vi "Connection Handler Worker.vi"(9 "Additional Data":variant, 10 "connection ID":T1, 11 "TCP Server Refnum":refnum<class "JKI TCP Server.lvclass">) -> ()   [LabVIEW 2020, in "CSM-TCP-Router.lvlib"]
uses:
  CSM-TCP-Router.lvlib
  <vilib>/addons/_JKI.lib/_JKI_lib_TCP_Server.llb/TCP Server Connection Session ID Cluster.ctl
  <vilib>/addons/_JKI.lib/_JKI_lib_TCP_Server.llb/JKI TCP Server.lvclass
  tcp-msg type.ctl
  <userlib>/_NEVSTOP/Communicable State Machine(CSM)/AdvanceAPI/CSM - Broadcast Message Type.ctl
  20ff867f-262a-4864-b042-c50abd455195.vi
  9f8653f6-ccbf-4dca-88e7-a4c531b7661f.vi
  bd168d05-2ccd-4f69-90c9-be1b4e621865.vi
  316abe05-dd11-44a4-98b3-32ea1594dc48.vi
  a7f8194b-54d4-448d-8a65-d0b66a8fd47c.vi
  8a9da1d4-9237-4126-a3a1-8a9d876b672d.vi
  66683ee4-8938-4a2b-95b9-1d8ed72716c9.vi
  <userlib>/_NEVSTOP/Communicable State Machine(CSM)/_Support/ChangeFlag/FlagInstance-CSMQ FGV.vi
  <userlib>/_NEVSTOP/Communicable State Machine(CSM)/_Support/ChangeFlag/FlagInstance-Broadcast Cache.vi
  <userlib>/_NEVSTOP/Communicable State Machine(CSM)/AdvanceAPI/CSM - Revert Arguments-Safe String.vi
  <userlib>/_NEVSTOP/Communicable State Machine(CSM)/AdvanceAPI/CSM - Make String Arguments Safe.vi
  <userlib>/_NEVSTOP/Communicable State Machine(CSM)/AdvanceAPI/CSM - Compact Multiple States.vi
  <userlib>/_NEVSTOP/Communicable State Machine(CSM)/_Support/ChangeFlag/ChangeFlag-Read.vi
  <userlib>/_NEVSTOP/Communicable State Machine(CSM)/AdvanceAPI/CSM - Keywords.vi
  <userlib>/_NEVSTOP/Communicable State Machine(CSM)/addons/API-String-Arugments-Support/_Support/Data To API String Arguments.vi
  <userlib>/_NEVSTOP/Communicable State Machine(CSM)/_Support/ChangeFlag/ChangeFlagDB.vi
  <userlib>/_NEVSTOP/Communicable State Machine(CSM)/_Support/BroadcastRegistry/HelperVI/Broadcast Item Key.vi
  <userlib>/_NEVSTOP/Communicable State Machine(CSM)/_Support/FGV-BroadcastRegistry/FGV-BroadcastRegistry(lvlibp).vi
  <userlib>/_NEVSTOP/Communicable State Machine(CSM)/addons/API-String-Arugments-Support/_Support/Query Data as API String Arguments(variant).vi
  <userlib>/_NEVSTOP/Communicable State Machine(CSM)/addons/API-String-Arugments-Support/_Support/Convert API String Arguments to Data(variant).vi
  <userlib>/_NEVSTOP/Communicable State Machine(CSM)/Communicable State Machine.lvlib
  <userlib>/_NEVSTOP/Communicable State Machine(CSM)/_csmHelper/API with lvcsm Support/CSM-Helper API with lvcsm Support.lvlib
  <userlib>/_NEVSTOP/Communicable State Machine(CSM)/_Shared/CSM Shared.lvlib
panel:
  out "State History":string
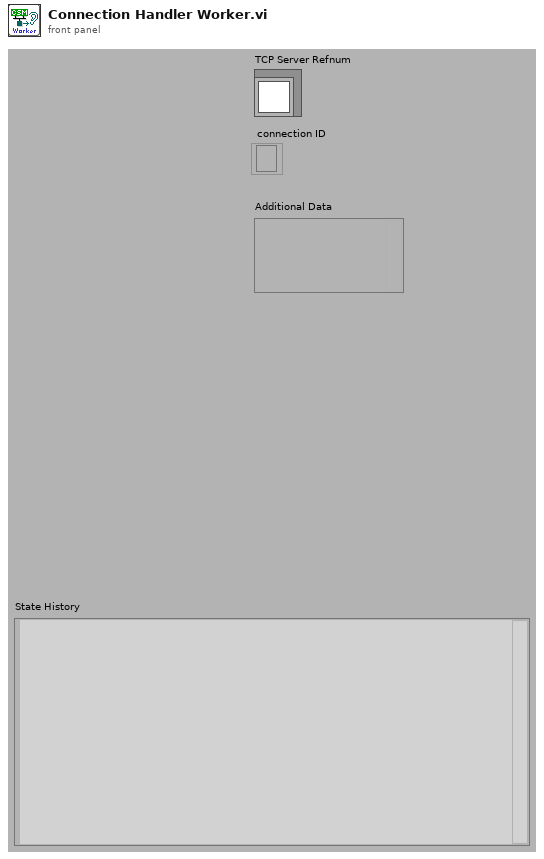
[diagram p1: front panel]
types:
  T1 = typedef "JKI TCP Server.lvclass/TCP Server Connection Session ID Cluster.ctl" = refnum<k5>
  T2 = typedef "CSM-TCP-Router.lvlib/tcp-msg type.ctl" = enum8{"info", "error", "cmd", "cmd-resp", "resp", "async-resp", "status", "interrupt"}
  T3 = typedef "Communicable State Machine.lvlib/CSM - Broadcast Message Type.ctl" = enum16{"<Null>", "Status", "Interrupt"}
  T4 = enum32{"Invalid", "Standard", "Closed", "Hidden", "Minimized", "Maximized"}
  T5 = enum32{"invalid app kind", "Development System", "Run Time System", "Student Edition", "Embedded LabVIEW", "Evaluation", "Custom"}
  T6 = typedef "Communicable State Machine.lvlib/_CSM_Response Source Message.ctl" = cluster{"‘State":string, "’Arguments":string, "’Error":errorcluster}
  T7 = cluster{"Target CSM":string, "Target State":string, "Register Type":T3}[]
  T8 = cluster{"Current VI Reference":refnum<vi>, "Close Panel on Exit?":bool}
  T9 = cluster{"Core":cluster{"Current VI Reference":refnum<vi>, "Close Panel on Exit?":bool}, "Your Boolean data":bool}
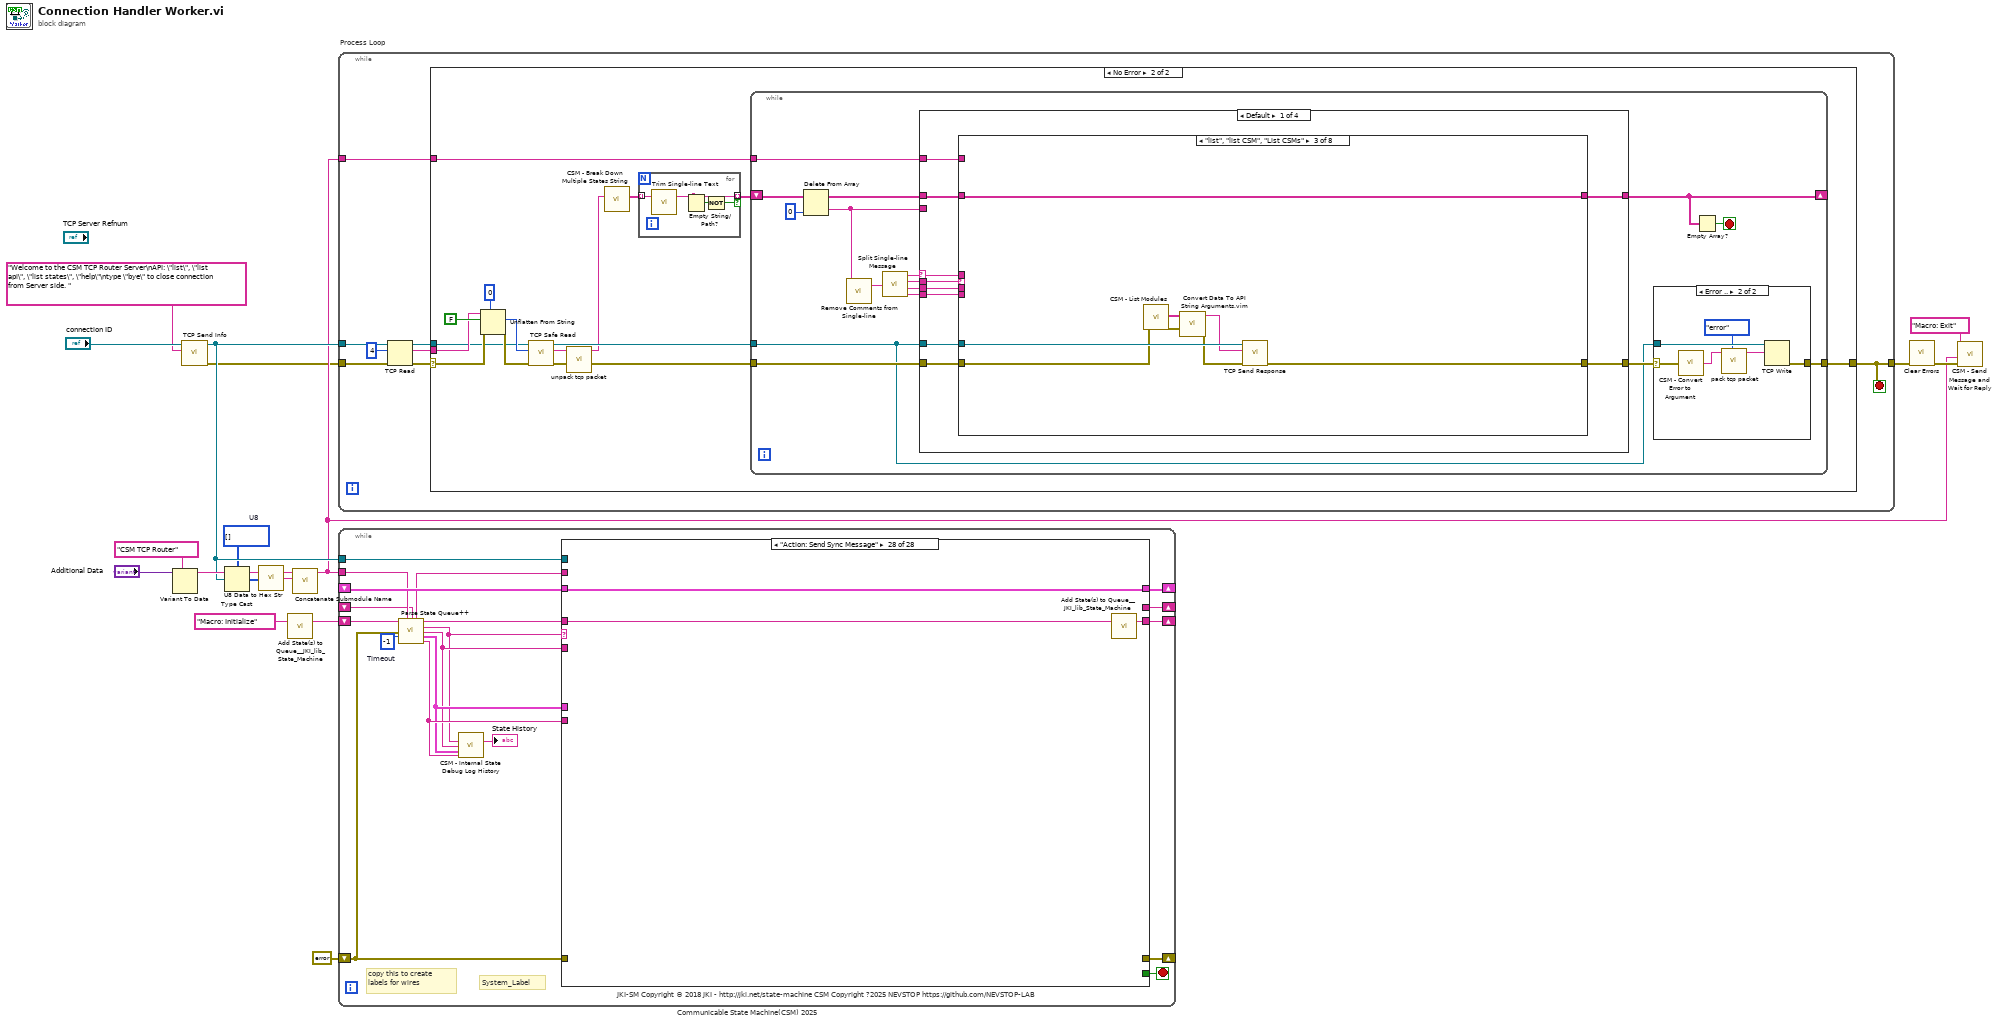
[diagram p0: block diagram]
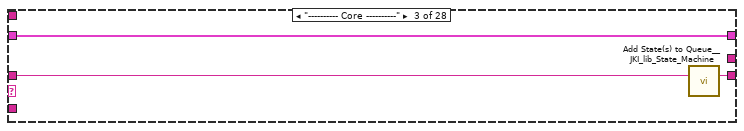
[diagram p4: hidden frame]
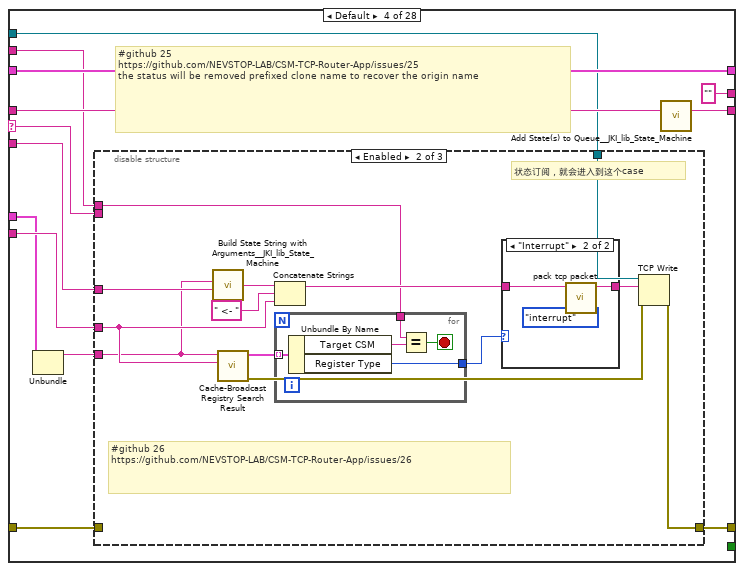
[diagram p5: hidden frame]
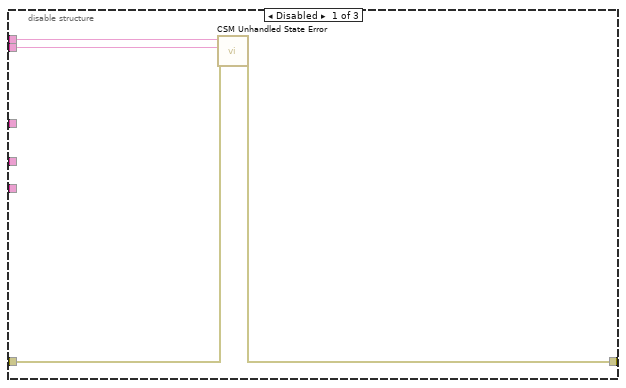
[diagram p6: hidden frame]
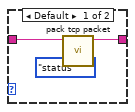
[diagram p7: hidden frame]
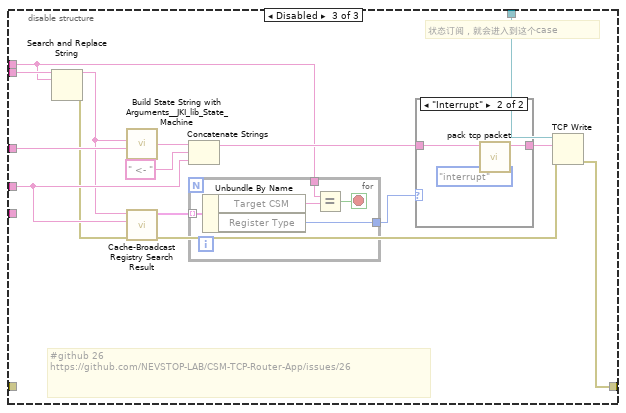
[diagram p8: hidden frame]
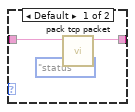
[diagram p9: hidden frame]
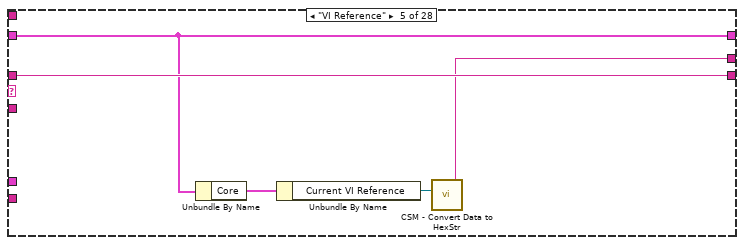
[diagram p10: hidden frame]
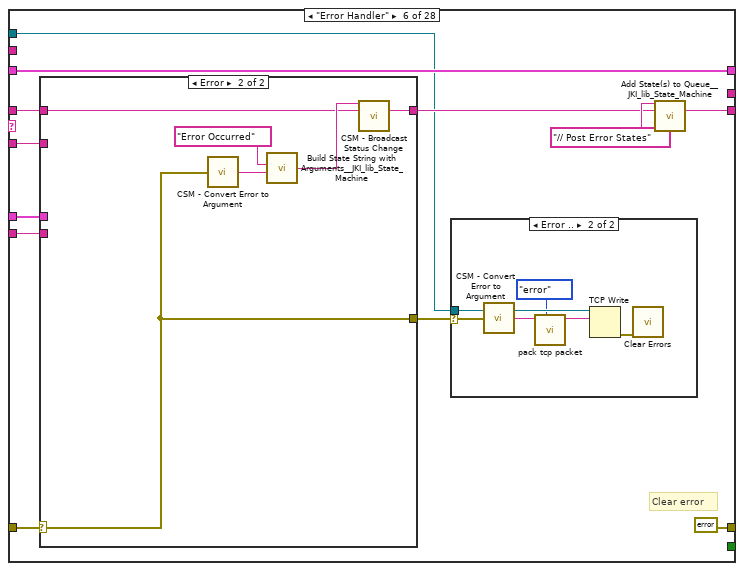
[diagram p11: hidden frame]
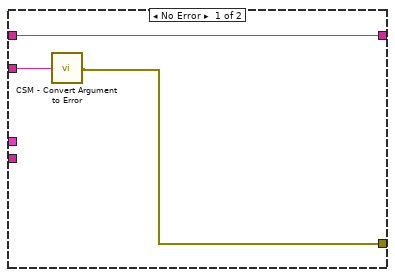
[diagram p13: hidden frame]
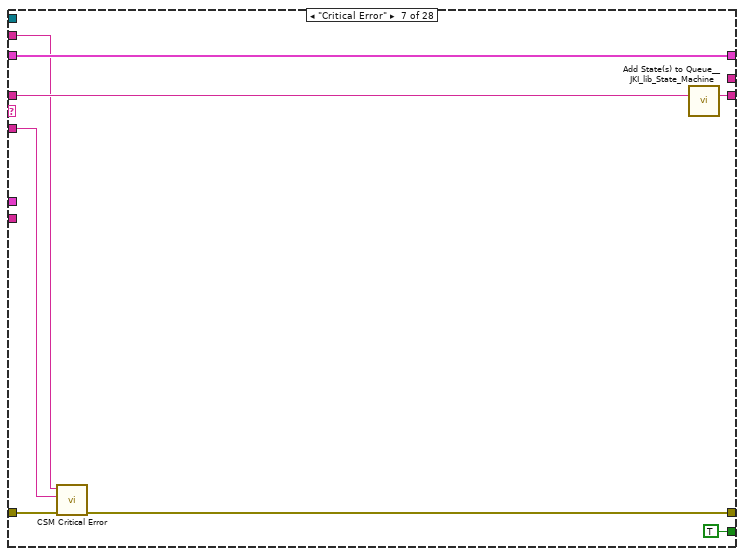
[diagram p14: hidden frame]
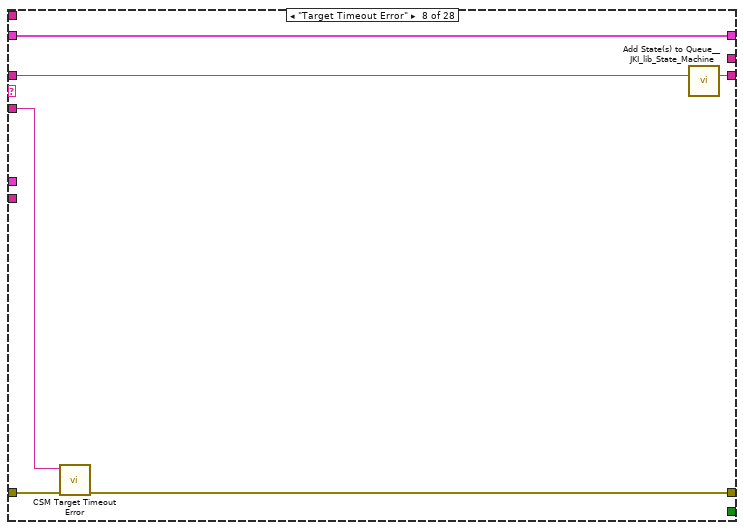
[diagram p15: hidden frame]
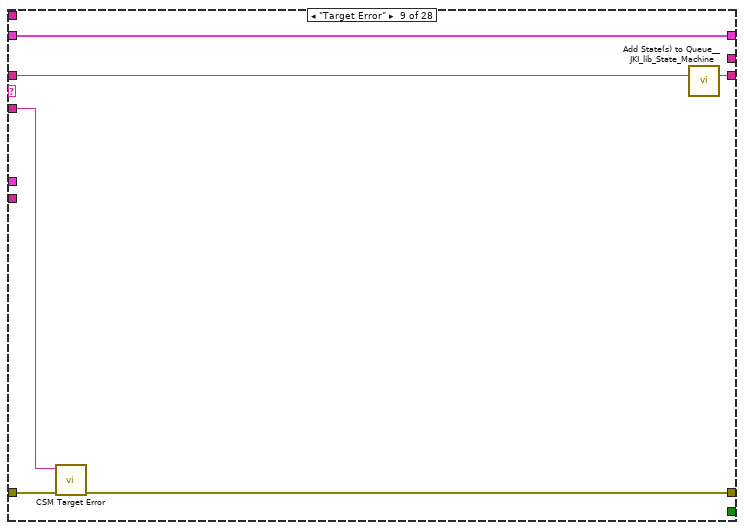
[diagram p16: hidden frame]
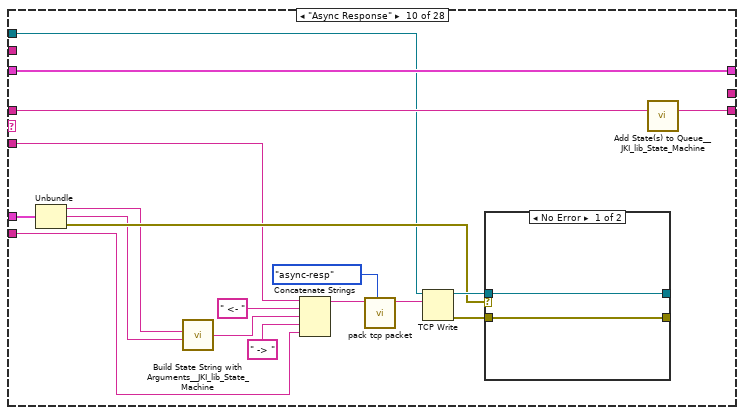
[diagram p17: hidden frame]
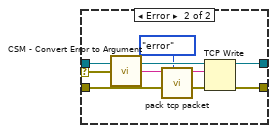
[diagram p18: hidden frame]
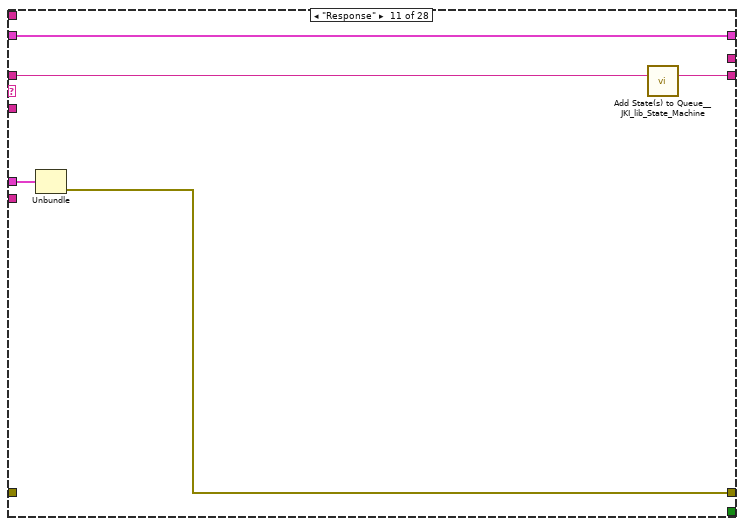
[diagram p19: hidden frame]
diagram:
  w5 = u8[] []  # U8
  n1 = Variant To Data(type="CSM TCP Router" ("Name(\"\" to use uuid)"), Variant="Additional Data") -> (data=w9:string)  [unwired: 1 in, 1 out]
  n2 = call "TCP Send Info.vi"("data in"="Welcome to the CSM TCP Router Server\nAPI: \"list\", \"list api\", \"list states\", \"help\"\ntype \"bye\" to close connection from Server side. ", "TCP Network Connection in"="connection ID") -> ("error out"=w2:errorcluster, "TCP Network Connection out"=w7:T1)  [unwired: 8 in]
  n3 = Type Cast(type=w5, x=w7) -> (*(type *) &x=w4:u8[])
  n4 = call <userlib>:"U8 Data to Hex Str.vi"("U8 Data[]"=w4) -> ("HEX String (0-9,A-F)"=w6:string)
  n5 = call <vilib>:"Add State(s) to Queue__JKI_lib_State_Machine.vi"("State(s) in (\"\")"="Macro: Initialize" ("Init States(\"Macro: Initialize\")")) -> ("States Out"=w15:string)  [unwired: 14 in]
  n6 = call <userlib>:"Concatenate Submodule Name.vi"("Module Name"=w6, "Group Name"=w9) -> ("Submodule Name"=w3:string)  [unwired: 9 in]
  n7 = while "Process Loop" {
    tunnel: w7 -> [w25]
    tunnel: [w21] -> w13
    tunnel: w3 -> [w20]
    tunnel: w2 -> [w18]
    stop <- w21 stop-if-true
    n8 = TCP Read(connection ID=w25, bytes to read=4, error in (no error)=w18) -> (connection ID out=w24:T1, data out=w22:string, error out=w23:errorcluster)  [unwired: 2 in]
    n9 = case shown="No Error" w23 {
      selector: w23 -> [w27 w37]
      tunnel: w24 -> [_ w30]
      tunnel: w22 -> [_ w38]
      tunnel: [w26 w44] -> w21
      tunnel: w20 -> [_ w41]
      frame Error {
        n10 = Unbundle By Name(w27) -> ("code"=w28:i32)
        n11 = case shown="56" w28 {
          tunnel: w27 -> [w29 _]
          tunnel: [w29 _] -> w26
          frame 0, Default {
          }
          frame 56 {
          }
        }
      }
      frame No Error {
        n12 = Unflatten From String(type=0, binary string=w38, data includes array or string size? (T)=FALSE, error in (no error)=w37) -> (value=w33:i32, error out=w36:errorcluster)  [unwired: 2 out]
        n13 = call "TCP Safe Read.vi"("error in (no error)"=w36, "bytes to read"=w33, "TCP Network Connection in"=w30) -> ("error out"=w35:errorcluster, "String"=w32:string, "TCP Network Connection out"=w34:refnum<k5>)  [unwired: 6 in]
        n14 = call "unpack tcp packet.vi"("TCP Pack"=w32) -> ("String"=w31:string)  [unwired: 9 in, 1 out]
        n15 = call <userlib>:"CSM - Break Down Multiple States String.vi"("States"=w31) -> ("Multiple States"=w43:string[])  [unwired: 10 in]
        n16 = for {
          tunnel: w43 -> [w48] mode=indexing
          tunnel: [w47] -> w42 mode=indexing if=w45
          n17 = call <userlib>:"Trim Single-line Text.vi"("single-line text"=w48) -> ("trimed text"=w47:string)  [unwired: 2 in]
          n18 = Empty String/Path?(string/path=w47) -> (empty?=w46:bool)
          n19 = Not(x=w46) -> (.not. x?=w45:bool)
        }
        n20 = while {
          tunnel: w34 -> [w51]
          tunnel: w35 -> [w64]
          tunnel: [w52] -> w44
          shift-right: [w54] -> _
          shift-left: w42 -> [w58]
          tunnel: w41 -> [w49]
          stop <- w55 stop-if-true
          n21 = Delete From Array(array=w58, index=0) -> (deleted portion=w50:string, array with subset deleted=w57:string[])  [unwired: 1 in]
          n22 = call <userlib>:"Remove Comments from Single-line.vi"("single-line text"=w50) -> ("single-line text without comments"=w63:string)  [unwired: 2 in]
          n23 = call <userlib>:"Split Single-line Message.vi"("single-line text"=w63) -> ("operator"=w62:string, "state"=w61:string, "args"=w60:string, "source/target"=w59:string)  [unwired: 6 in]
          n24 = case shown="Default" w62 {
            selector: w62 -> [w75 _ _ _]
            tunnel: w51 -> [w81 w192 w196 w267]
            tunnel: [w80 w191 w200 w271] -> w53
            tunnel: w64 -> [w79 w184 w198 w269]
            tunnel: w61 -> [w78 w186 w195 w266]
            tunnel: w60 -> [w77 w185 w194 w265]
            tunnel: w59 -> [w76 w187 w193 w264]
            tunnel: [w74 w189 w199 w270] -> w54
            tunnel: w57 -> [w73 w189 w199 w270]
            tunnel: w50 -> [_ _ _ _]
            tunnel: w49 -> [w72 w188 w197 w268]
            frame Default {
              n25 = case shown="\"list\", \"list CSM\", \"List CSMs\"" w78 {
                selector: w78 -> [w89 _ _ _ _ _ _ _]
                tunnel: w81 -> [w92 w97 w107 w120 w133 w146 w160 w180]
                tunnel: [w91 errorcluster {"status"=TRUE, "code"=0, "source"=""} ("error out") w102 w119 w132 w145 w162 w181] -> w80
                tunnel: w79 -> [w84 w98 w106 _ _ _ w161 w178]
                tunnel: w77 -> [w90 _ _ w115 w128 w141 _ _]
                tunnel: w76 -> [_ _ _ _ _ _ _ _]
                tunnel: w75 -> [_ _ _ _ _ _ _ _]
                tunnel: [w88 w95 w101 w118 w131 w144 w168 w182] -> w74
                tunnel: w73 -> [w88 w95 w101 w118 w131 w144 w168 w182]
                tunnel: w72 -> [_ _ _ w114 w127 w140 w163 _]
                frame Default {
                  n26 = call <vilib>:"Build State String with Arguments__JKI_lib_State_Machine.vi"("Arguments (\"\")"=w90, "State"=w89) -> ("State with Arguments"=w85:string)  [unwired: 4 in]
                  n27 = Format Into String(format string="You typed \"%s\", which is not recognized as a command", w85) -> (resulting string=w86:string)  [unwired: 2 in, 1 out]
                  n28 = call "pack tcp packet.vi"("tcp-message-type"=tcp-msg_type."error", "String"=w86) -> ("TCP Pack"=w83:string)  [unwired: 9 in]
                  n29 = TCP Write(connection ID=w92, data in=w83, error in (no error)=w84) -> (error out=w91:errorcluster)  [unwired: 1 in, 2 out]
                }
                frame "bye", "exit", "quit" {
                  n30 = call "TCP Send Info.vi"("error in (no error)"=w98, "data in"="Good bye.\r\n", "TCP Network Connection in"=w97) -> ("error out"=w94:errorcluster, "TCP Network Connection out"=w93:T1)  [unwired: 7 in]
                  n31 = TCP Close Connection(connection ID=w93, error in (no error)=w94) -> ()  [unwired: 1 in, 2 out]
                }
                frame "list", "list CSM", "List CSMs" {
                  n32 = call <userlib>:"CSM - List Modules.vi"("Error In"=w106) -> ("error out"=w104:errorcluster, "Module Names"=w105:string[])  [unwired: 9 in]
                  n33 = call "Convert Data To API String Arguments.vim"("error in (no error)"=w104, "Data"=w105) -> ("error out"=w103:errorcluster, "API String"=w100:string)  [unwired: 6 in]
                  n34 = call "TCP Send Response.vi"("error in (no error)"=w103, "Response"=w100, "connection ID"=w107) -> ("error out"=w102:errorcluster)  [unwired: 7 in, 1 out]
                }
                frame "list API", "list interface" {
                  n35 = call <userlib>:"CSM - Check If Module Exists.vi"("CSM Name"=w115) -> ("error out"=w117:errorcluster, "Exist?"=w112:bool, "CSM Name (Dup)"=w116:string)  [unwired: 8 in]
                  n36 = call "Error If Module Not Exist.vi"("Error in"=w117, "Module Exist?"=w112) -> ("Error out"=w113:errorcluster)  [unwired: 9 in]
                  n37 = call <userlib>:"Read CSM API with lvcsm Support.vi"("Current Module (\"\" to Generate an ID)"=w114, "error in (no error)"=w113, "CSM Name"=w116) -> ("error out"=w110:errorcluster, "CSMAPI List"=w109:string[])  [unwired: 7 in]
                  n38 = call "Convert Data To API String Arguments.vim"("error in (no error)"=w110, "Data"=w109) -> ("error out"=w111:errorcluster, "API String"=w108:string)  [unwired: 6 in]
                  n39 = call "TCP Send Response.vi"("error in (no error)"=w111, "Response"=w108, "connection ID"=w120) -> ("error out"=w119:errorcluster)  [unwired: 7 in, 1 out]
                }
                frame "List State", "List States" {
                  n40 = call <userlib>:"CSM - Check If Module Exists.vi"("CSM Name"=w128) -> ("error out"=w130:errorcluster, "Exist?"=w125:bool, "CSM Name (Dup)"=w129:string)  [unwired: 8 in]
                  n41 = call "Error If Module Not Exist.vi"("Error in"=w130, "Module Exist?"=w125) -> ("Error out"=w126:errorcluster)  [unwired: 9 in]
                  n42 = call <userlib>:"Read CSM States with lvcsm Support.vi"("Current Module (\"\" to Generate an ID)"=w127, "error in (no error)"=w126, "CSM Name"=w129) -> ("error out"=w121:errorcluster, "CSMAPI List"=w122:string[])  [unwired: 7 in]
                  n43 = call "Convert Data To API String Arguments.vim"("error in (no error)"=w121, "Data"=w122) -> ("error out"=w124:errorcluster, "API String"=w123:string)  [unwired: 6 in]
                  n44 = call "TCP Send Response.vi"("error in (no error)"=w124, "Response"=w123, "connection ID"=w133) -> ("error out"=w132:errorcluster)  [unwired: 7 in, 1 out]
                }
                frame "help" {
                  n45 = call <userlib>:"CSM - Check If Module Exists.vi"("CSM Name"=w141) -> ("error out"=w143:errorcluster, "Exist?"=w138:bool, "CSM Name (Dup)"=w142:string)  [unwired: 8 in]
                  n46 = call "Error If Module Not Exist.vi"("Error in"=w143, "Module Exist?"=w138) -> ("Error out"=w139:errorcluster)  [unwired: 9 in]
                  n47 = disable-structure shown="Enabled" {
                    disable-tunnel: w139 -> [w153 w158]
                    disable-tunnel: w142 -> [w152 w157]
                    disable-tunnel: [w150 w155] -> w135
                    disable-tunnel: [w148 w154] -> w134
                    disable-tunnel: w140 -> [w147 w156]
                    frame Disabled {
                      n48 = call <userlib>:"CSM - Module VI Reference.vi"("Current Module (\"\" to Generate an ID)"=w147, "error in (no error)"=w153, "CSM Name"=w152) -> ("error out"=w151:errorcluster, "CSM Module VIRef"=w149:refnum<vi>)  [unwired: 7 in]
                      n49 = property class="VI"(reference=w149, error in=w151) -> (error out=w150:errorcluster, "Description"=w148:string)  [unwired: 1 out]
                    }
                    frame Enabled {
                      n50 = call "Read CSM Doc.vi"("Current Module(\"\" to generate a ID)"=w156, "error in (no error)"=w158, "CSM Name"=w157) -> ("Error out"=w155:errorcluster, "CSM Doc"=w154:string)  [unwired: 7 in]
                    }
                  }
                  n51 = call "Convert Data To API String Arguments.vim"("error in (no error)"=w135, "Data"=w134) -> ("error out"=w137:errorcluster, "API String"=w136:string)  [unwired: 6 in]
                  n52 = call "TCP Send Response.vi"("error in (no error)"=w137, "Response"=w136, "connection ID"=w146) -> ("error out"=w145:errorcluster)  [unwired: 7 in, 1 out]
                }
                frame "Refresh lvcsm" {
                  n53 = call <userlib>:"CSM - List Modules.vi"("Error In"=w161) -> ("error out"=w167:errorcluster, "Module Names"=w166:string[])  [unwired: 9 in]
                  n54 = for {
                    tunnel: w167 -> [w177]
                    tunnel: w166 -> [w170] mode=indexing
                    tunnel: [w172] -> w165 mode=indexing
                    tunnel: w163 -> [w171]
                    n55 = call <userlib>:"Read CSM States with lvcsm Support.vi"("Current Module (\"\" to Generate an ID)"=w171, "error in (no error)"=w177, "Force? (F)"=TRUE ("Force?(F)"), "CSM Name"=w170) -> ("error out"=w176:errorcluster)  [unwired: 6 in, 1 out]
                    n56 = call <userlib>:"Read CSM API with lvcsm Support.vi"("Current Module (\"\" to Generate an ID)"=w171, "error in (no error)"=w176, "Force? (F)"=TRUE ("Force?(F)"), "CSM Name"=w170) -> ("error out"=w173:errorcluster)  [unwired: 6 in, 1 out]
                    n57 = call "Read CSM Doc.vi"("Current Module(\"\" to generate a ID)"=w171, "error in (no error)"=w173, "Force?(F)"=TRUE, "CSM Name"=w170) -> ("Error out"=w172:errorcluster)  [unwired: 6 in, 1 out]
                  }
                  n58 = Merge Errors(w165) -> (w164:errorcluster)
                  n59 = call "TCP Send Response.vi"("error in (no error)"=w164, "Response"="", "connection ID"=w160) -> ("error out"=w162:errorcluster)  [unwired: 7 in, 1 out]
                }
                frame "ping" {
                  n60 = call "TCP Send Response.vi"("error in (no error)"=w178, "Response"="pong", "connection ID"=w180) -> ("error out"=w181:errorcluster)  [unwired: 7 in, 1 out]
                }
              }
            }
            frame "-@" {
              n61 = call <userlib>:"CSM - Send Message and Wait for Reply.vi"("Current Module (\"\" to Generate an ID)"=w188, "Error In (No Error)"=w184, "Target Module"=w187, "Arguments (\"\")"=w185, "State"=w186) -> ("error out"=w183:errorcluster, "Response"=w190:string)  [unwired: 4 in, 1 out]
              n62 = call "TCP Send Response.vi"("error in (no error)"=w183, "Response"=w190, "connection ID"=w192) -> ("error out"=w191:errorcluster)  [unwired: 7 in, 1 out]
            }
            frame "->" {
              # "#github 25\nhttps://github.com/NEVSTOP-LAB/CSM-TCP-Router-App/issues/25\nthe status will be prefixed the clone name"
              n63 = case shown="\"<register as status>\"" w193 {
                selector: w193 -> [_ _ _ _ w254]
                tunnel: [w204 w217 w230 w243 w260] -> w200
                tunnel: w198 -> [_ _ _ _ w259]
                tunnel: w197 -> [w203 w215 w227 w240 w258]
                tunnel: w196 -> [w206 w219 w232 w245 w257]
                tunnel: w195 -> [w211 w223 w236 w249 w256]
                tunnel: w194 -> [w212 w224 w237 w250 w255]
                frame "<unregister>" {
                  n64 = call <userlib>:"Parse Unregister Message.vi"("State"=w211, "Module Name"=w203, "Args"=w212) -> ("Target"=w209:string, "Source"=w210:string, "Status"=w208:string, "Api"=w202:string)  [unwired: 8 in, 1 out]
                  n65 = Concatenate Strings(w203, w202) -> (w201:string)
                  n66 = call <userlib>:"CSM - Unregister Broadcast.vi"("CSM Name(Empty for Broadcast Event)"=w209, "Source CSM Name (* as Default)"=w210, "Trigger"=w208, "API (\"*\" as Default)"=w201) -> ("error out"=w205:errorcluster)  [unwired: 10 in, 1 out]
                  n67 = call "TCP Send Command Respone.vi"("error in (no error)"=w205, "Response"="done", "connection ID"=w206) -> ("error out"=w204:errorcluster)  [unwired: 7 in, 1 out]
                }
                frame "<register>" {
                  n68 = call <userlib>:"Parse Register Message.vi"("State"=w223, "Module Name"=w215, "Args"=w224) -> ("Target"=w221:string, "Source"=w222:string, "Status"=w220:string, "Api"=w214:string)  [unwired: 8 in, 1 out]
                  n69 = Concatenate Strings(w215, w214) -> (w213:string)
                  n70 = call <userlib>:"CSM - Register Broadcast.vi"("CSM Name(Empty for Broadcast Event)"=w221, "Source CSM Name (* as Default)"=w222, "Trigger"=w220, "API (If \"\", Same as Trigger)"=w213) -> ("error out"=w218:errorcluster)  [unwired: 10 in, 1 out]
                  n71 = call "TCP Send Command Respone.vi"("error in (no error)"=w218, "Response"="done", "connection ID"=w219) -> ("error out"=w217:errorcluster)  [unwired: 7 in, 1 out]
                }
                frame "<register as status>" {
                  n72 = call <userlib>:"Parse Register Message.vi"("State"=w236, "Module Name"=w227, "Args"=w237) -> ("Target"=w234:string, "Source"=w235:string, "Status"=w233:string, "Api"=w226:string)  [unwired: 8 in, 1 out]
                  n73 = Concatenate Strings(w227, w226) -> (w225:string)
                  n74 = call <userlib>:"CSM - Register Broadcast.vi"("CSM Name(Empty for Broadcast Event)"=w234, "Source CSM Name (* as Default)"=w235, "Trigger"=w233, "API (If \"\", Same as Trigger)"=w225, "Priority (No Change)"=CSM_-_Broadcast_Message_Type."Status") -> ("error out"=w231:errorcluster)  [unwired: 9 in, 1 out]
                  n75 = call "TCP Send Command Respone.vi"("error in (no error)"=w231, "Response"="done", "connection ID"=w232) -> ("error out"=w230:errorcluster)  [unwired: 7 in, 1 out]
                }
                frame "<register as interrupt>" {
                  n76 = call <userlib>:"Parse Register Message.vi"("State"=w249, "Module Name"=w240, "Args"=w250) -> ("Target"=w247:string, "Source"=w248:string, "Status"=w246:string, "Api"=w239:string)  [unwired: 8 in, 1 out]
                  n77 = Concatenate Strings(w240, w239) -> (w238:string)
                  n78 = call <userlib>:"CSM - Register Broadcast.vi"("CSM Name(Empty for Broadcast Event)"=w247, "Source CSM Name (* as Default)"=w248, "Trigger"=w246, "API (If \"\", Same as Trigger)"=w238, "Priority (No Change)"=CSM_-_Broadcast_Message_Type."Interrupt") -> ("error out"=w244:errorcluster)  [unwired: 9 in, 1 out]
                  n79 = call "TCP Send Command Respone.vi"("error in (no error)"=w244, "Response"="done", "connection ID"=w245) -> ("error out"=w243:errorcluster)  [unwired: 7 in, 1 out]
                }
                frame Default {
                  n80 = call <userlib>:"CSM - Request CSM to Post Message.vi"("Module Name"=w258, "Target Module (\"\" By Default)"=w254, "Arguments (\"\")"=w255, "State"=w256) -> ("error out"=w251:errorcluster)  [unwired: 7 in]
                  n81 = Merge Errors(w259, w251) -> (w252:errorcluster)
                  n82 = call "TCP Send Command Respone.vi"("error in (no error)"=w252, "Response"="Message posted", "connection ID"=w257) -> ("error out"=w260:errorcluster)  [unwired: 7 in, 1 out]
                }
              }
            }
            frame "->|" {
              n83 = call <userlib>:"CSM - Post Message.vi"("Current Module (\"\" to Generate an ID)"=w268, "Target Module"=w264, "Arguments (\"\")"=w265, "State"=w266) -> ("error out"=w262:errorcluster)  [unwired: 7 in]
              n84 = call "Synchronize Data Flow.vim"("input 2"=w269, "input 1"=w262) -> ("output 2"=w263:errorcluster)  [unwired: 2 in, 3 out]
              n85 = call "TCP Send Command Respone.vi"("error in (no error)"=w263, "Response"="No-Rep Message Posted", "connection ID"=w267) -> ("error out"=w271:errorcluster)  [unwired: 7 in, 1 out]
            }
          }
          n86 = case shown="Error .." w53 {
            selector: w53 -> [w65 w68]
            tunnel: w51 -> [_ w71]
            tunnel: [w65 w70] -> w52
            frame No Error {
            }
            frame Error {
              n87 = call <userlib>:"CSM - Convert Error to Argument.vi"("Error"=w68) -> ("Argument"=w69:string)  [unwired: 4 in]
              n88 = call "pack tcp packet.vi"("tcp-message-type"=tcp-msg_type."error", "String"=w69) -> ("TCP Pack"=w67:string)  [unwired: 9 in]
              n89 = TCP Write(connection ID=w71, data in=w67) -> (error out=w70:errorcluster)  [unwired: 2 in, 2 out]
            }
          }
          n90 = Empty Array?(array=w54) -> (empty?=w55:bool)
        }
      }
    }
  }
  n91 = while "Communicable State Machine(CSM) 2025" {
    shift-right: [w285] -> _
    shift-left: _ -> [w284]
    shift-right: [w288] -> _
    shift-left: errorcluster {"status"=FALSE, "code"=0, "source"=""} ("error out") -> [w274]
    shift-right: [w287] -> _
    shift-left: w15 -> [w289]
    tunnel: w3 -> [w281]
    shift-right: [w282] -> _
    shift-left: _ -> [w276]
    tunnel: w7 -> [w272]
    stop <- w286 stop-if-true
    w283 = -1  # Timeout
    # "copy this to create labels for wires"
    # "System_Label"
    # "JKI-SM Copyright © 2018 JKI - http://jki.net/state-machine CSM Copyright ?2025 NEVSTOP https://github.com/NEVSTOP-LAB"
    n92 = call <userlib>:"Parse State Queue++.vi"("State Queue"=w289, "Name (\"\" to Use UUID)"=w281, "Response Arguments"=w276, "Previous Error"=w274, "Dequeue (1 ms)"=w283) -> ("Name Used"=w275:string, "Remaining States"=w290:string, "Current State"=w277:string, "Arguments"=w278:string, "Additional Information"=w279:T6, "Source CSM"=w280:string)  [unwired: 5 in]
    n93 = call <userlib>:"CSM - Internal State Debug Log History.vi"("State"=w277, "Arguments (\"\")"=w278, ">> Response Source Message >>"=w279, "Source (\"\")"=w280) -> ("Debug Log"=→"State History":string)  [unwired: 11 in]
    n94 = case shown="\"Action: Send Sync Message\"" w277 {
      selector: w277 -> [_ _ _ w305 _ _ _ _ _ _ _ _ _ _ _ _ _ _ _ _ _ _ _ _ _ _ _ _]
      tunnel: w290 -> [w291 w294 w297 w308 w369 w375 w403 w409 w415 w432 w447 w451 w463 w467 w470 w475 w481 w486 w488 w493 w496 w500 w504 w506 w509 w513 w518 w521]
      tunnel: w278 -> [_ _ _ w301 _ w374 w397 w406 w412 w424 _ _ _ _ _ _ w476 w485 _ _ _ _ _ _ _ w511 _ _]
      tunnel: w284 -> [w292 w293 w295 w306 w366 w380 w401 w407 w413 w433 w448 w450 w457 w465 w468 _ w480 w484 w487 w489 w494 w498 w502 w505 w508 w512 w516 w519]
      tunnel: [_ _ _ w310 _ errorcluster {"status"=FALSE, "code"=0, "source"=""} ("error out") w404 w405 w411 _ w445 _ _ _ _ _ w477 w482 _ w490 _ _ _ _ _ _ _ _] -> w288
      tunnel: w274 -> [_ _ _ w309 _ w378 w399 w410 w416 _ _ _ _ _ _ _ _ _ _ _ _ _ _ _ _ _ _ _]
      tunnel: [w291 w294 w296 w307 w369 w376 w402 w408 w414 w434 w449 w451 w462 w466 w469 w474 w481 w486 w488 w492 w495 w499 w503 w506 w509 w513 w517 w520] -> w287
      tunnel: [_ _ _ _ _ _ TRUE _ _ _ _ _ _ TRUE _ _ _ _ _ _ _ _ _ _ _ _ _ _] -> w286
      tunnel: [w292 w293 w295 w306 w366 w380 w401 w407 w413 w433 w448 w450 w461 w465 w468 w473 w479 w483 w487 w489 w494 w498 w502 w505 w508 w512 w516 w519] -> w285
      tunnel: w280 -> [_ _ _ w300 _ w373 _ _ _ w417 _ _ _ _ _ _ _ _ _ _ _ _ _ _ _ _ _ _]
      tunnel: w279 -> [_ _ _ w299 _ w372 _ _ _ w431 w446 _ _ _ _ _ _ _ _ _ _ _ _ _ _ _ _ _]
      tunnel: [_ _ _ "" w365 _ _ _ _ _ _ _ _ _ _ _ w478 _ _ _ _ _ _ _ "API1 Response" w510 _ _] -> w282
      tunnel: w275 -> [_ _ _ w303 _ _ w398 _ _ _ _ _ _ _ _ _ _ _ _ _ _ _ _ _ _ _ _ _]
      tunnel: w272 -> [_ _ _ w302 _ w370 _ _ _ w425 _ _ _ _ _ _ _ _ _ _ _ _ _ _ _ _ _ _]
      frame "", "Idle" {
      }
      frame "CSM Documentation" {
      }
      frame "---------- Core ----------" {
        n95 = call <vilib>:"Add State(s) to Queue__JKI_lib_State_Machine.vi"("State(s) in (\"\")"=w297) -> ("States Out"=w296:string)  [unwired: 14 in]
      }
      frame Default {
        # "#github 25\nhttps://github.com/NEVSTOP-LAB/CSM-TCP-Router-App/issues/25\nthe status will be removed prefixed clone name to recover the origin name"
        n96 = Unbundle(w299) -> ("‘State"=w298:string)  [unwired: 2 out]
        n97 = disable-structure shown="Enabled" {
          disable-tunnel: [w314 w321 w347] -> w310
          disable-tunnel: w309 -> [w313 _ _]
          disable-tunnel: w305 -> [w312 _ w343]
          disable-tunnel: w303 -> [w311 w317 w340]
          disable-tunnel: w302 -> [_ w324 w350]
          disable-tunnel: w301 -> [_ w323 w349]
          disable-tunnel: w300 -> [_ w320 w346]
          disable-tunnel: w298 -> [_ w315 _]
          frame Disabled {
            n98 = call <userlib>:"CSM Unhandled State Error.vi"("error in (no error)"=w313, "Undefined State"=w312, "CSM Name"=w311) -> ("error out"=w314:errorcluster)  [unwired: 8 in]
          }
          frame Enabled {
            # "#github 26\nhttps://github.com/NEVSTOP-LAB/CSM-TCP-Router-App/issues/26"
            # "状态订阅，就会进入到这个case"
            n99 = call <vilib>:"Build State String with Arguments__JKI_lib_State_Machine.vi"("Arguments (\"\")"=w323, "State"=w315) -> ("State with Arguments"=w322:string)  [unwired: 4 in]
            n100 = call <userlib>:"Cache-Broadcast Registry Search Result.vi"("CSM Name"=w320, "Broadcast State"=w315) -> ("error out"=w319:errorcluster, "Array"=w318:T7)  [unwired: 8 in]
            n101 = Concatenate Strings(w322, " <- " ("string"), w320) -> (w326:string)
            n102 = for {
              tunnel: w318 -> [w332] mode=indexing
              tunnel: w317 -> [w330]
              tunnel: [w329] -> w316
              stop <- w328 stop-if-true
              n103 = Unbundle By Name(w332) -> ("Target CSM"=w331:string, "Register Type"=w329:T3)
              n104 = Equal?(x=w330, y=w331) -> (x = y?=w328:bool)
            }
            n105 = case shown="\"Interrupt\"" w316 {
              tunnel: [w334 w338] -> w327
              tunnel: w326 -> [w335 w337]
              frame Default {
                n106 = call "pack tcp packet.vi"("tcp-message-type"=tcp-msg_type."status", "String"=w335) -> ("TCP Pack"=w334:string)  [unwired: 9 in]
              }
              frame "Interrupt" {
                n107 = call "pack tcp packet.vi"("tcp-message-type"=tcp-msg_type."interrupt", "String"=w337) -> ("TCP Pack"=w338:string)  [unwired: 9 in]
              }
            }
            n108 = TCP Write(connection ID=w324, data in=w327, error in (no error)=w319) -> (error out=w321:errorcluster)  [unwired: 1 in, 2 out]
          }
          frame Disabled {
            # "#github 26\nhttps://github.com/NEVSTOP-LAB/CSM-TCP-Router-App/issues/26"
            # "状态订阅，就会进入到这个case"
            n109 = Search and Replace String(input string=w343, search string=w340) -> (result string=w342:string, error out=w344:errorcluster)  [unwired: 6 in, 2 out]
            n110 = call <vilib>:"Build State String with Arguments__JKI_lib_State_Machine.vi"("Arguments (\"\")"=w349, "State"=w342) -> ("State with Arguments"=w348:string)  [unwired: 4 in]
            n111 = call <userlib>:"Cache-Broadcast Registry Search Result.vi"("error in (no error)"=w344, "CSM Name"=w346, "Broadcast State"=w342) -> ("error out"=w345:errorcluster, "Array"=w341:T7)  [unwired: 7 in]
            n112 = Concatenate Strings(w348, " <- " ("string"), w346) -> (w352:string)
            n113 = for {
              tunnel: w341 -> [w358] mode=indexing
              tunnel: w340 -> [w356]
              tunnel: [w355] -> w339
              stop <- w354 stop-if-true
              n114 = Unbundle By Name(w358) -> ("Target CSM"=w357:string, "Register Type"=w355:T3)
              n115 = Equal?(x=w356, y=w357) -> (x = y?=w354:bool)
            }
            n116 = case shown="\"Interrupt\"" w339 {
              tunnel: [w360 w364] -> w353
              tunnel: w352 -> [w361 w363]
              frame Default {
                n117 = call "pack tcp packet.vi"("tcp-message-type"=tcp-msg_type."status", "String"=w361) -> ("TCP Pack"=w360:string)  [unwired: 9 in]
              }
              frame "Interrupt" {
                n118 = call "pack tcp packet.vi"("tcp-message-type"=tcp-msg_type."interrupt", "String"=w363) -> ("TCP Pack"=w364:string)  [unwired: 9 in]
              }
            }
            n119 = TCP Write(connection ID=w350, data in=w353, error in (no error)=w345) -> (error out=w347:errorcluster)  [unwired: 1 in, 2 out]
          }
        }
        n120 = call <vilib>:"Add State(s) to Queue__JKI_lib_State_Machine.vi"("State(s) in (\"\")"=w308) -> ("States Out"=w307:string)  [unwired: 14 in]
      }
      frame "VI Reference" {
        n121 = Unbundle By Name(w366) -> ("Core"=w368:T8)
        n122 = Unbundle By Name(w368) -> ("Current VI Reference"=w367:refnum<vi>)
        n123 = call <userlib>:"CSM - Convert Data to HexStr.vi"("Variant"=w367) -> ("HEX String (0-9,A-F)"=w365:string)  [unwired: 8 in]
      }
      frame "Error Handler" {
        # "Clear error"
        n124 = case shown="Error" w378 {
          selector: w378 -> [_ w391]
          tunnel: [w390 w393] -> w377
          tunnel: w375 -> [w390 w392]
          tunnel: w374 -> [w389 _]
          tunnel: w373 -> [_ _]
          tunnel: w372 -> [_ _]
          tunnel: [w388 w391] -> w371
          frame No Error {
            n125 = call <userlib>:"CSM - Convert Argument to Error.vi"("Argument"=w389) -> ("Error"=w388:errorcluster)  [unwired: 4 in]
          }
          frame Error {
            n126 = call <userlib>:"CSM - Convert Error to Argument.vi"("Error"=w391) -> ("Argument"=w395:string)  [unwired: 4 in]
            n127 = call <vilib>:"Build State String with Arguments__JKI_lib_State_Machine.vi"("Arguments (\"\")"=w395, "State"="Error Occurred" ("Status with Arguments")) -> ("State with Arguments"=w394:string)  [unwired: 4 in]
            n128 = call <userlib>:"CSM - Broadcast Status Change.vi"("Status With Arguments"=w394, "State Queue"=w392) -> ("Remaining States"=w393:string)  [unwired: 13 in]
          }
        }
        n129 = case shown="Error .." w371 {
          selector: w371 -> [_ w385]
          tunnel: w370 -> [_ w387]
          frame No Error {
          }
          frame Error {
            n130 = call <userlib>:"CSM - Convert Error to Argument.vi"("Error"=w385) -> ("Argument"=w384:string)  [unwired: 4 in]
            n131 = call "pack tcp packet.vi"("tcp-message-type"=tcp-msg_type."error", "String"=w384) -> ("TCP Pack"=w383:string)  [unwired: 9 in]
            n132 = TCP Write(connection ID=w387, data in=w383) -> (error out=w386:errorcluster)  [unwired: 2 in, 2 out]
            n133 = call <vilib>:"Clear Errors.vi"("error in (no error)"=w386) -> ()  [unwired: 5 in, 2 out]
          }
        }
        n134 = call <vilib>:"Add State(s) to Queue__JKI_lib_State_Machine.vi"("State(s) in Front (\"\")"="// Post Error States", "State(s) in (\"\")"=w377) -> ("States Out"=w376:string)  [unwired: 13 in]
      }
      frame "Critical Error" {
        n135 = call <userlib>:"CSM Critical Error.vi"("error in (no error)"=w399, "Arugments (As Reason)"=w397, "CSM Name"=w398) -> ("error out"=w404:errorcluster)  [unwired: 8 in]
        n136 = call <vilib>:"Add State(s) to Queue__JKI_lib_State_Machine.vi"("State(s) in (\"\")"=w403) -> ("States Out"=w402:string)  [unwired: 14 in]
      }
      frame "Target Timeout Error" {
        n137 = call <userlib>:"CSM Target Timeout Error.vi"("error in (no error)"=w410, "Arguments (As CSM Name)"=w406) -> ("error out"=w405:errorcluster)  [unwired: 9 in]
        n138 = call <vilib>:"Add State(s) to Queue__JKI_lib_State_Machine.vi"("State(s) in (\"\")"=w409) -> ("States Out"=w408:string)  [unwired: 14 in]
      }
      frame "Target Error" {
        n139 = call <userlib>:"CSM Target Error.vi"("error in (no error)"=w416, "Arguments (As CSM Name)"=w412) -> ("error out"=w411:errorcluster)  [unwired: 9 in]
        n140 = call <vilib>:"Add State(s) to Queue__JKI_lib_State_Machine.vi"("State(s) in (\"\")"=w415) -> ("States Out"=w414:string)  [unwired: 14 in]
      }
      frame "Async Response" {
        n141 = Unbundle(w431) -> ("‘State"=w421:string, "’Arguments"=w420:string, "’Error"=w426:errorcluster)
        n142 = call <vilib>:"Build State String with Arguments__JKI_lib_State_Machine.vi"("Arguments (\"\")"=w420, "State"=w421) -> ("State with Arguments"=w419:string)  [unwired: 4 in]
        n143 = Concatenate Strings(w424, " <- " ("string"), w419, " -> " ("string"), w417) -> (w423:string)
        n144 = call "pack tcp packet.vi"("tcp-message-type"=tcp-msg_type."async-resp", "String"=w423) -> ("TCP Pack"=w430:string)  [unwired: 9 in]
        n145 = TCP Write(connection ID=w425, data in=w430) -> (connection ID out=w429:T1, error out=w428:errorcluster)  [unwired: 2 in, 1 out]
        n146 = case shown="No Error" w426 {
          selector: w426 -> [_ w441]
          tunnel: w428 -> [w436 w444]
          tunnel: w429 -> [w435 w443]
          tunnel: [w436 w442] -> _
          tunnel: [w435 w439] -> _
          frame No Error {
          }
          frame Error {
            n147 = call <userlib>:"CSM - Convert Error to Argument.vi"("Error"=w441) -> ("Argument"=w440:string)  [unwired: 4 in]
            n148 = call "pack tcp packet.vi"("tcp-message-type"=tcp-msg_type."error", "String"=w440) -> ("TCP Pack"=w438:string)  [unwired: 9 in]
            n149 = TCP Write(connection ID=w443, data in=w438, error in (no error)=w444) -> (connection ID out=w439:T1, error out=w442:errorcluster)  [unwired: 1 in, 1 out]
          }
        }
        n150 = call <vilib>:"Add State(s) to Queue__JKI_lib_State_Machine.vi"("State(s) in (\"\")"=w432) -> ("States Out"=w434:string)  [unwired: 14 in]
      }
      frame "Response" {
        n151 = Unbundle(w446) -> ("’Error"=w445:errorcluster)  [unwired: 2 out]
        n152 = call <vilib>:"Add State(s) to Queue__JKI_lib_State_Machine.vi"("State(s) in (\"\")"=w447) -> ("States Out"=w449:string)  [unwired: 14 in]
      }
      frame "Async Message Posted" {
      }
      frame "Initialize Core Data" {
        # "originally closed?"
        # "exe?"
        # "If panel starts closed or is an EXE, then close it when we exit"
        n153 = property class="VI"() -> ("FP.State"=w454:T4)  [unwired: 2 in, 2 out]
        n154 = property class="App"() -> ("App.Kind"=w460:T5)  [unwired: 2 in, 2 out]
        n155 = control-ref of="Current VI Reference"() -> (w455:refnum<vi>)
        n156 = Equal?(x=w454, y=T4."Closed" ("Front Panel Window:State")) -> (x = y?=w452:bool)
        n157 = Equal?(x=w460, y=T5."Run Time System" ("Application:Kind")) -> (x = y?=w458:bool)
        n158 = Or(x=w452, y=w458) -> (x .or. y?=w456:bool)
        n159 = Bundle By Name(cluster=w457, "Core.Current VI Reference"=w455, "Core.Close Panel on Exit?"=w456) -> (w461:T9)
        n160 = call <vilib>:"Add State(s) to Queue__JKI_lib_State_Machine.vi"("State(s) in (\"\")"=w463) -> ("States Out"=w462:string)  [unwired: 14 in]
      }
      frame "Exit" {
        n161 = call <vilib>:"Add State(s) to Queue__JKI_lib_State_Machine.vi"("State(s) in (\"\")"=w467) -> ("States Out"=w466:string)  [unwired: 14 in]
      }
      frame "---------- Data ----------" {
        n162 = call <vilib>:"Add State(s) to Queue__JKI_lib_State_Machine.vi"("State(s) in (\"\")"=w470) -> ("States Out"=w469:string)  [unwired: 14 in]
      }
      frame "Data: Initialize" {
        w471 = T8 {"Current VI Reference"=refnum, "Close Panel on Exit?"=FALSE}  # Core
        w472 = TRUE  # Your Boolean data
        n163 = Bundle("Core"=w471, "Your Boolean data"=w472) -> (w473:T9)  [unwired: 1 in]
        n164 = call <vilib>:"Add State(s) to Queue__JKI_lib_State_Machine.vi"("State(s) in (\"\")"=w475) -> ("States Out"=w474:string)  [unwired: 14 in]
      }
      frame "Data: Get Configuration", "Data: Get Internal Data" {
        n165 = call "Query Data as API String Arguments.vim"("Name"=w476, "Cluster Data"=w480) -> ("error"=w477:errorcluster, "API String"=w478:string, "Cluster Data (dup)"=w479:T9)  [unwired: 7 in]
      }
      frame "Data: Set Configuration" {
        n166 = call "Convert API String Arguments to Data.vim"("Reference Type"=w484, "API String"=w485) -> ("error out"=w482:errorcluster, "Data"=w483:T9)  [unwired: 6 in]
      }
      frame "Data: Update Indicators" {
      }
      frame "Data: Cleanup" {
        n167 = Unbundle By Name(w489) -> ("Core.Current VI Reference"=w491:refnum<vi>)
        n168 = Close Reference(reference=w491) -> (error out=w490:errorcluster)  [unwired: 1 in]
        n169 = call <vilib>:"Add State(s) to Queue__JKI_lib_State_Machine.vi"("State(s) in (\"\")"=w493) -> ("States Out"=w492:string)  [unwired: 14 in]
      }
      frame "---------- Macro ----------" {
        n170 = call <vilib>:"Add State(s) to Queue__JKI_lib_State_Machine.vi"("State(s) in (\"\")"=w496) -> ("States Out"=w495:string)  [unwired: 14 in]
      }
      frame "Macro: Initialize" {
        n171 = call <vilib>:"Add State(s) to Queue__JKI_lib_State_Machine.vi"("State(s) in Front (\"\")"="Data: Initialize\nInitialize Core Data\nData: Update Indicators", "State(s) in (\"\")"=w500) -> ("States Out"=w499:string)  [unwired: 13 in]
      }
      frame "Macro: Exit" {
        n172 = call <vilib>:"Add State(s) to Queue__JKI_lib_State_Machine.vi"("State(s) in Front (\"\")"="Data: Cleanup\nExit", "State(s) in (\"\")"=w504) -> ("States Out"=w503:string)  [unwired: 13 in]
      }
      frame "---------- API ----------" {
      }
      frame "API: API1" {
      }
      frame "API: API2" {
        # "unpack Hex String  to Variant\nif complex parameter is needed."
        n173 = call <userlib>:"CSM - Convert HexStr to Data.vi"("HEX String"=w511) -> ()  [unwired: 7 in, 2 out]
        n174 = disable-structure shown="Enabled" {
          disable-tunnel: [w514 "API2 Response"] -> w510
          frame Disabled {
            # "pack variant to hexstr \nif complex response is needed."
            # "complex Response"
            n175 = call <userlib>:"CSM - Convert Data to HexStr.vi"() -> ("HEX String (0-9,A-F)"=w514:string)  [unwired: 9 in]
          }
          frame Enabled {
          }
        }
      }
      frame "---------- Action ----------" {
        n176 = call <vilib>:"Add State(s) to Queue__JKI_lib_State_Machine.vi"("State(s) in (\"\")"=w518) -> ("States Out"=w517:string)  [unwired: 14 in]
      }
      frame "Action: Send Sync Message" {
        n177 = call <vilib>:"Add State(s) to Queue__JKI_lib_State_Machine.vi"("State(s) in (\"\")"=w521) -> ("States Out"=w520:string)  [unwired: 14 in]
      }
    }
  }
  n178 = call <vilib>:"Clear Errors.vi"("error in (no error)"=w13) -> ("error out"=w12:errorcluster)  [unwired: 5 in, 1 out]
  n179 = call <userlib>:"CSM - Send Message and Wait for Reply.vi"("Error In (No Error)"=w12, "Target Module"=w3, "State"="Macro: Exit") -> ()  [unwired: 6 in, 3 out]
